vi "Tank Simulator - Volume of liquid.vi"(6 "history length":i32, 7 "VC Handle":T1=-1, 8 "error in":errorcluster, 9 "cmd":enum16{"init", "get", "set"}(ring)=enum."get", 10 "value in":dbl format="%.2f", 11 "var name":string) -> (0 "error out":errorcluster, 2 "value out":dbl format="%.2f", 3 "var name out":string, 5 "VC Handle out":T1=-1)   [LabVIEW 2021]
doc: "Handler for <B>Volume</B> variable.\n\n::: CalcExpress Toolkit :::\nCopyright (c) 2000-2026 Konstantin Shifershteyn. All rights reserved."
uses:
  vi.lib/addons/CalcExpress/cetypes.llb/VarMan Variable Context Handle.ctl
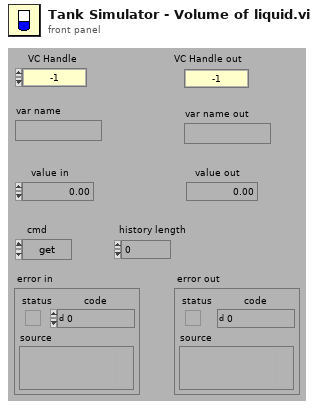
[diagram p1: front panel]
types:
  T1 = typedef "VarMan Variable Context Handle.ctl" = i32
  T2 = enum16{"create", "destroy", "set value", "get value"}
  T3 = enum32{"nop", "create", "destroy", "reset", "get info", "config"}
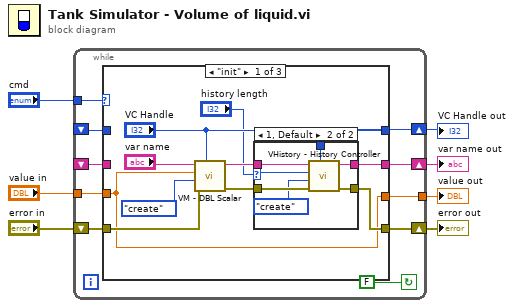
[diagram p0: block diagram]
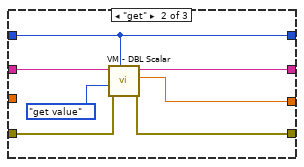
[diagram p3: hidden frame]
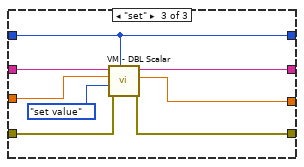
[diagram p4: hidden frame]
diagram:
  n1 = while {
    tunnel: [w9] -> w4
    tunnel: "value in" -> [w14]
    shift-left: "error in" -> [w13]
    shift-right: [w12] -> w3
    shift-left: _ -> [w11]
    shift-right: [w16] -> w1
    shift-left: _ -> [w10]
    shift-right: [w15] -> w2
    tunnel: "cmd" -> [w17]
    stop <- FALSE continue-if-true
    n2 = case shown="\"init\"" w17 {
      tunnel: [w22 w43 w51] -> w16
      tunnel: ["VC Handle" w38 w46] -> w15
      tunnel: w14 -> [w18 _ w45]
      tunnel: w13 -> [w26 w42 w50]
      tunnel: [w19 w41 w49] -> w12
      tunnel: w11 -> [_ w39 w47]
      tunnel: w10 -> [_ w38 w46]
      tunnel: [w18 w37 w44] -> w9
      frame "init" {
        n3 = call "VM - DBL Scalar.vi"("VC Handle"="VC Handle", "error in"=w26, "cmd"=T2."create", "value in"=w18, "name_spec"="var name") -> ("error out"=w21:errorcluster, "dup name_spec"=w24:string)  [unwired: 1 in, 4 out]
        n4 = case shown="1, Default" "history length" {
          selector: "history length" -> [_ w32]
          tunnel: w24 -> [w29 w36]
          tunnel: "VC Handle" -> [_ w35]
          tunnel: [w29 w34] -> w22
          tunnel: w21 -> [w28 w33]
          tunnel: [w28 w31] -> w19
          frame 0 {
          }
          frame 1, Default {
            n5 = call "VHistory - History Controller.vi"("VC Handle"=w35, "error in"=w33, "cmd (nop:default)"=T3."create", "history length"=w32, "name_spec"=w36) -> ("error out"=w31:errorcluster, "dup name_spec"=w34:string)  [unwired: 3 in, 2 out]
          }
        }
      }
      frame "get" {
        n6 = call "VM - DBL Scalar.vi"("VC Handle"=w38, "error in"=w42, "cmd"=T2."get value", "name_spec"=w39) -> ("error out"=w41:errorcluster, "value out"=w37:dbl, "dup name_spec"=w43:string)  [unwired: 2 in, 3 out]
      }
      frame "set" {
        n7 = call "VM - DBL Scalar.vi"("VC Handle"=w46, "error in"=w50, "cmd"=T2."set value", "value in"=w45, "name_spec"=w47) -> ("error out"=w49:errorcluster, "value out"=w44:dbl, "dup name_spec"=w51:string)  [unwired: 1 in, 3 out]
      }
    }
  }
  "value out" <- w4
  "error out" <- w3
  "VC Handle out" <- w2
  "var name out" <- w1
